vi "Close Modbus.vi"(8 "error in (no error)":errorcluster, 11 "Modbus_Master in":refnum<class "Modbus_Master.lvclass">) -> (0 "error out":errorcluster, 3 "Modbus_Master out":refnum<class "Modbus_Master.lvclass">)   [LabVIEW 2021, in "Modbus_Master.lvclass"]
uses:
  Modbus_Master.lvclass
  <vilib>/NI/Modbus Library/API/Master/Modbus Master.lvclass
  Modbus_Master.lvclass/Modbus_Master.ctl
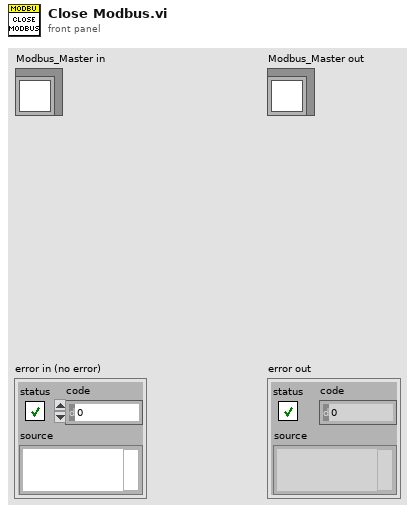
[diagram p1: front panel]
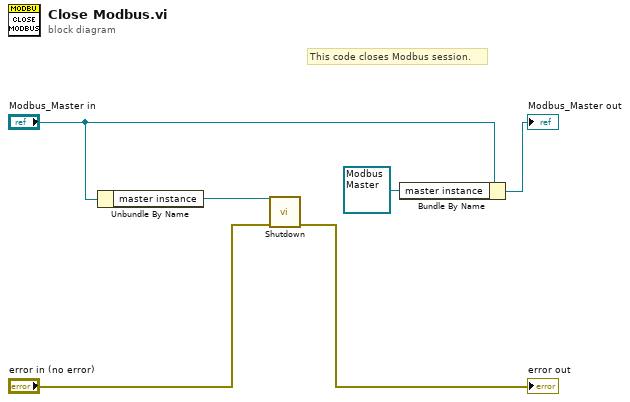
[diagram p0: block diagram]
diagram:
  # "This code closes Modbus session."
  n1 = Unbundle By Name("Modbus_Master in") -> ("master instance"=w1:refnum<class "Modbus Master.lvclass">)
  n2 = call-dynamic "Shutdown.vi"("error in"="error in (no error)", "Modbus master in"=w1) -> ("error out"=→"error out":errorcluster)  [unwired: 9 in]
  n3 = Bundle By Name(cluster="Modbus_Master in", "master instance"=refnum<class "Modbus Master.lvclass"> refnum) -> (→"Modbus_Master out":refnum<class "Modbus_Master.lvclass">)
